vi "user process.vi"(8 "error in":errorcluster, 10 "MotionModule runtime in":refnum<class "MotionModule runtime.lvclass">, 11 "Parameters to process":T2) -> (0 "error out":errorcluster, 2 "MotionModule runtime Out":refnum<class "MotionModule runtime.lvclass">, 3 "Results from processing":T1)   [LabVIEW 2017, in "MotionModule runtime.lvclass"]
uses:
  MotionModule runtime.lvclass
  parameter user data.ctl
  result user data.ctl
  MotionModule runtime.lvclass/MotionModule runtime.ctl
  Utilities/StateMachine.ctl
  Utilities/Controlword_Commands.ctl
  Utilities/MoveMode.ctl
  SoftmotionClass/SoftmotionAxis/SoftmotionAxis.lvclass
  Utilities/WordManipulationLibrary.lvlib
  Utilities/Bit Manipulation.lvlib
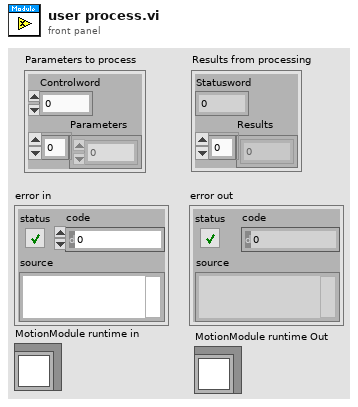
[diagram p1: front panel]
types:
  T1 = typedef "MotionModule runtime.lvclass/result user data.ctl" = cluster{"Statusword":u16, "Results":dbl[]}
  T2 = typedef "MotionModule runtime.lvclass/parameter user data.ctl" = cluster{"Controlword":u16, "Parameters":dbl[]}
  T3 = typedef "WordManipulationLibrary.lvlib/StateMachine.ctl" = enum16{"Start", "Not Ready to Switch On", "Switch On Disabled", "Ready to Switch On", "Switched On", "Operation enable", "Quick Stop Active", "Fault Reaction Active", "Fault"}
  T4 = typedef "WordManipulationLibrary.lvlib/Controlword_Commands.ctl" = enum16{"Shutdown", "Switch On", "Disable Voltage", "Quick Stop", "Disable Op", "Enable Op", "Fault Reset", "Error"}
  T5 = typedef "WordManipulationLibrary.lvlib/MoveMode.ctl" = enum16{"Reserved", "Profile Position Mode", "Velocity Mode", "Profile Velocity Mode", "Profile Torque Mode", "Reserved 2", "Reference Mode", "Interpolated Position Mode", "Skip"}
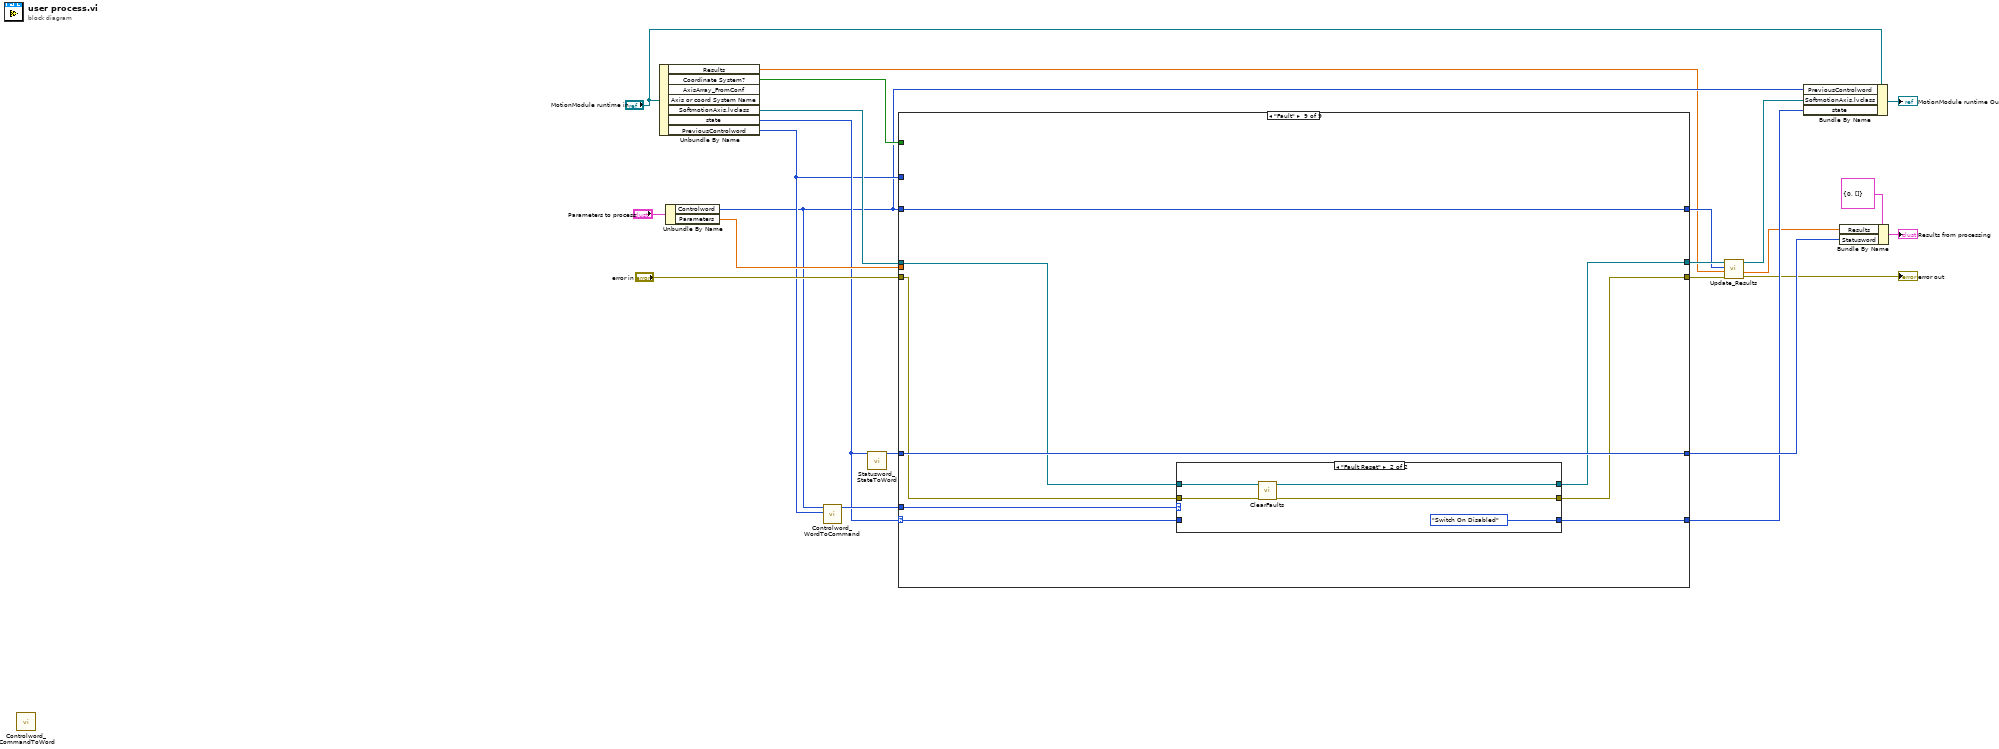
[diagram p0: block diagram]
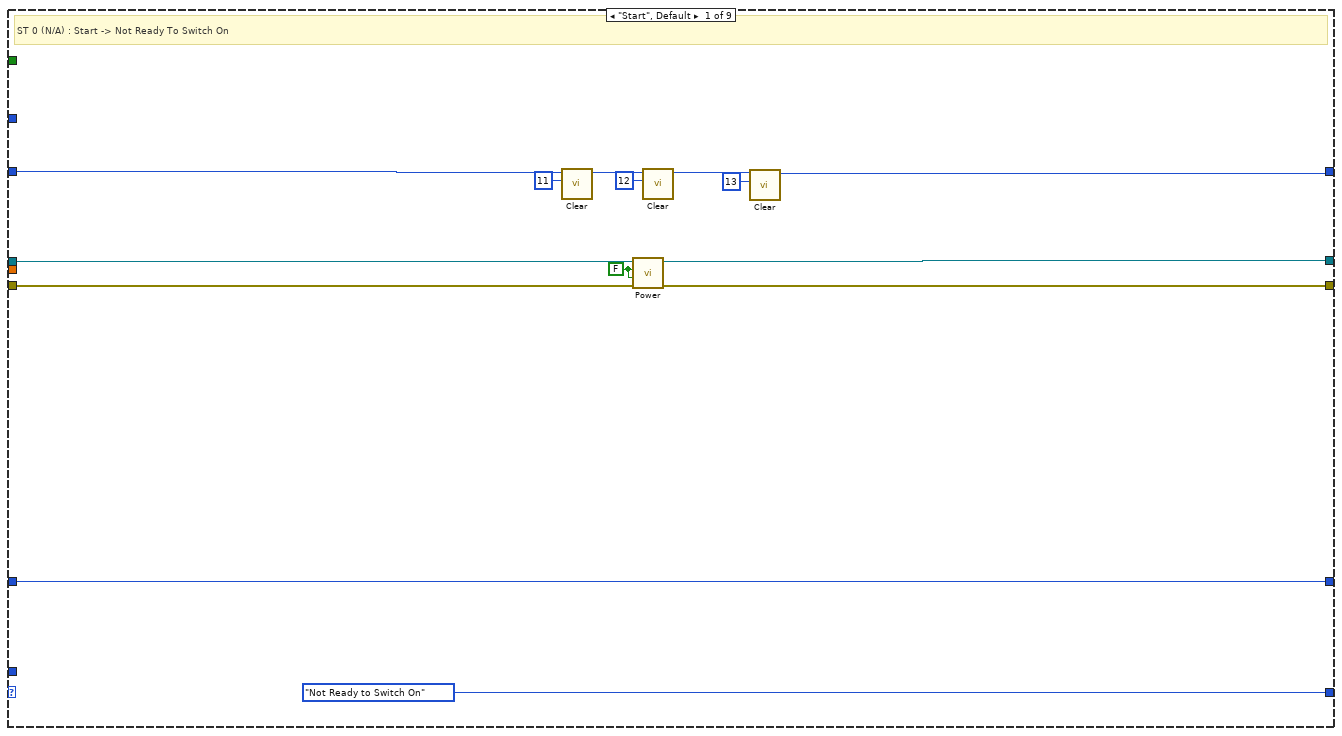
[diagram p2: hidden frame]
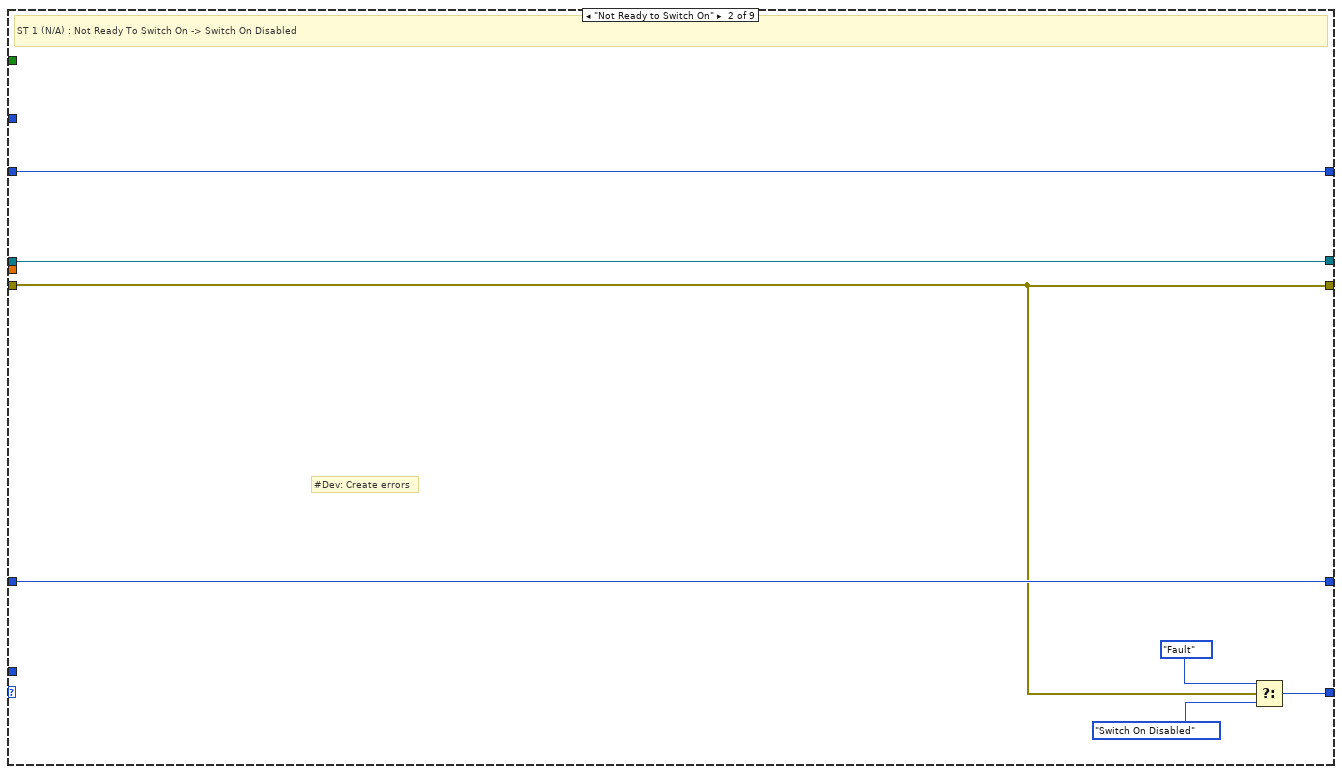
[diagram p3: hidden frame]
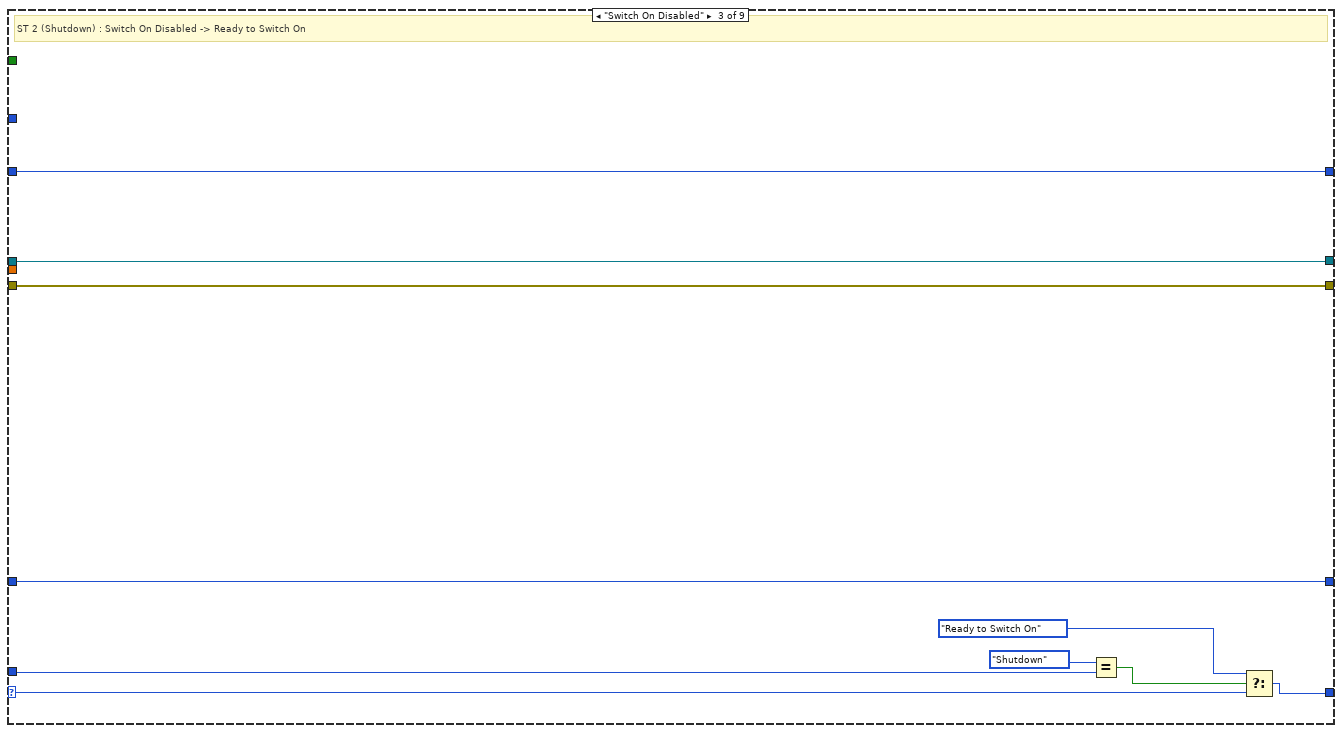
[diagram p4: hidden frame]
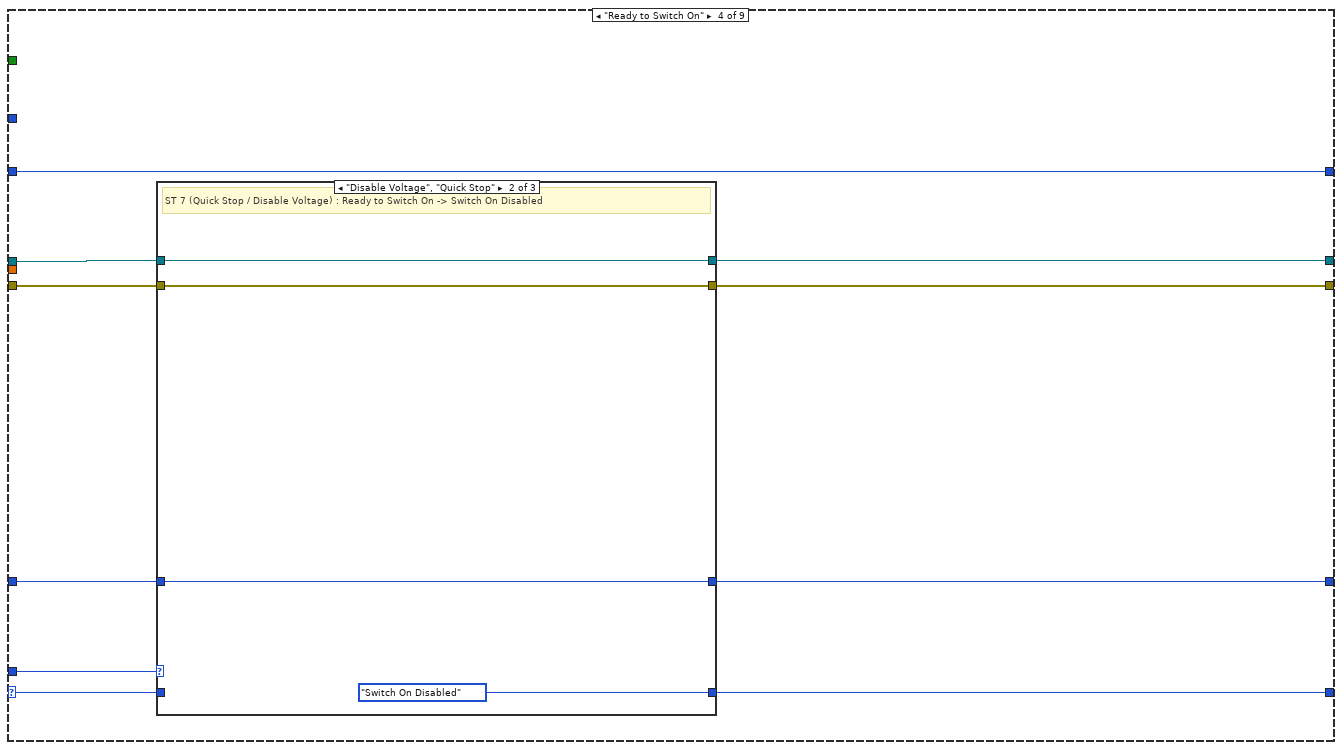
[diagram p5: hidden frame]
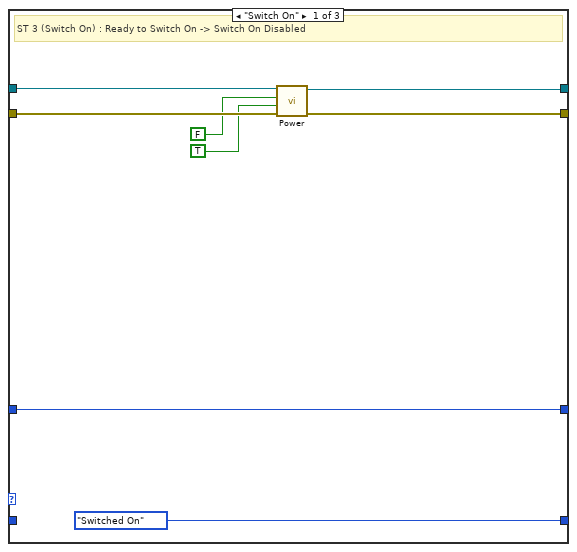
[diagram p6: hidden frame]
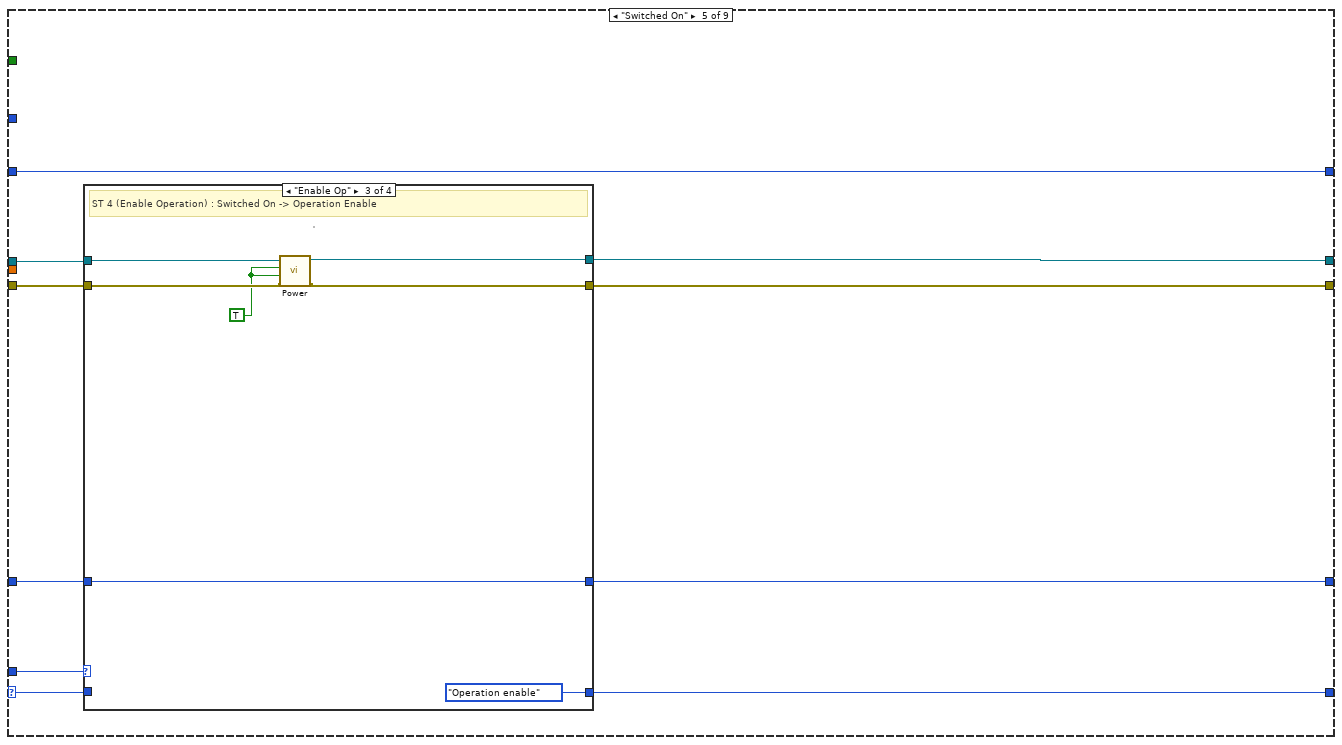
[diagram p8: hidden frame]
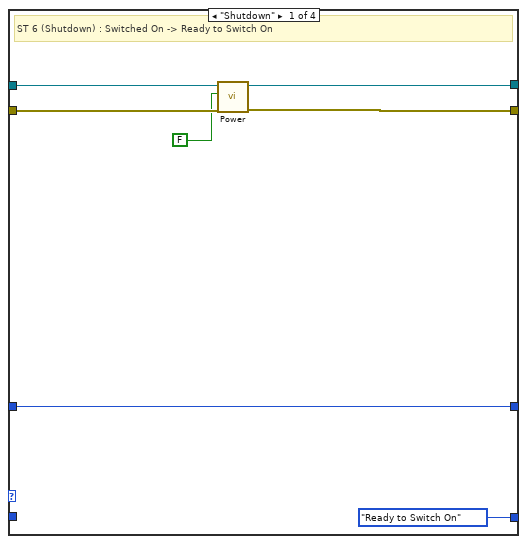
[diagram p9: hidden frame]
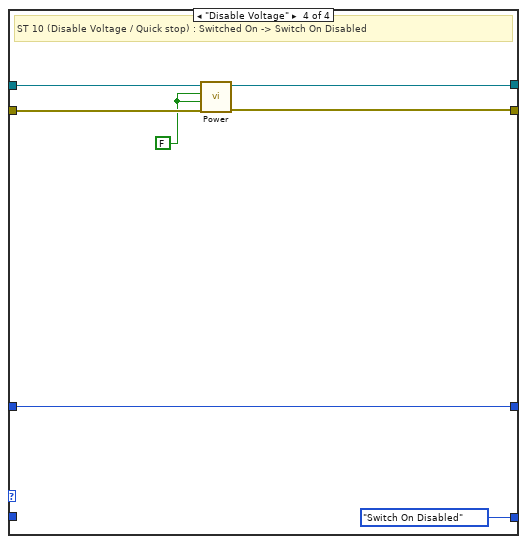
[diagram p11: hidden frame]
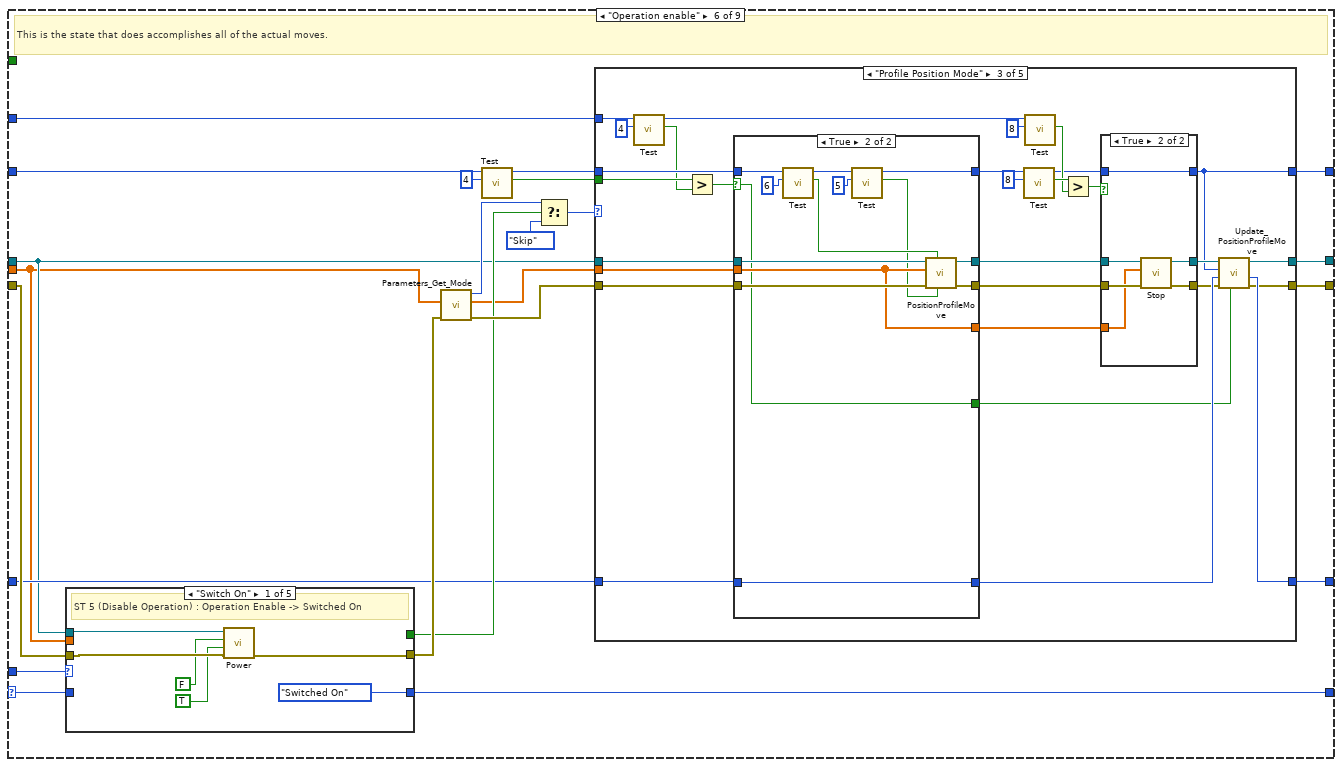
[diagram p12: hidden frame]
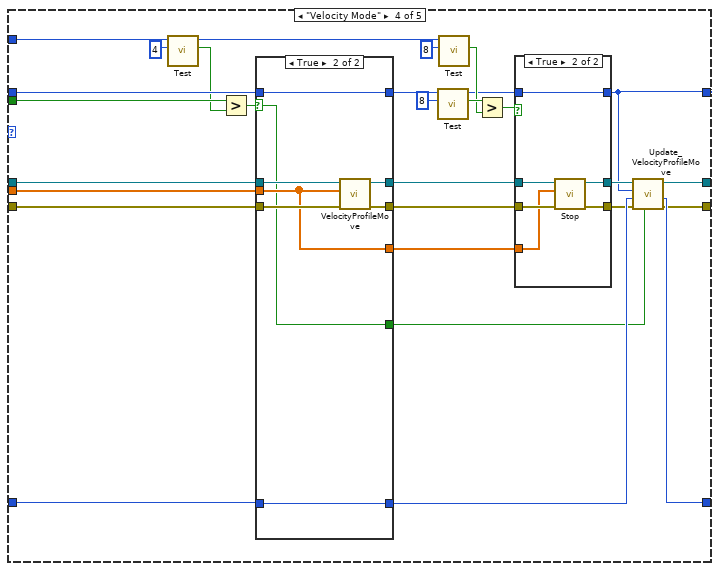
[diagram p17: hidden frame]
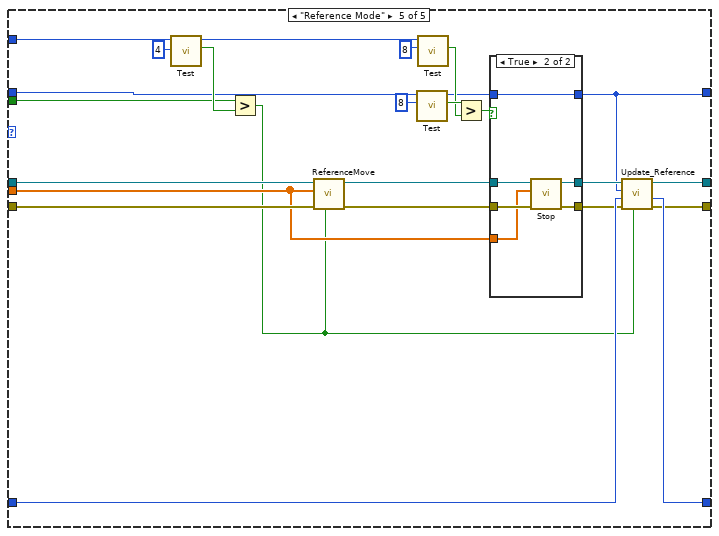
[diagram p20: hidden frame]
diagram:
  n1 = call "Controlword_CommandToWord.vi"() -> ()  [unwired: 11 in, 1 out]
  n2 = Unbundle By Name("MotionModule runtime in") -> ("Results"=w4:dbl[], "Coordinate System?"=w9:bool, "SoftmotionAxis.lvclass"=w18:refnum<class "SoftmotionAxis.lvclass">, "state"=w12:T3, "PreviousControlword"=w10:u16)  [unwired: 2 out]
  n3 = Unbundle By Name("Parameters to process") -> ("Controlword"=w8:u16, "Parameters"=w20:dbl[])
  n4 = call "Controlword_WordToCommand.vi"("Previous Controlword"=w10, "Controlword"=w8) -> ("Device Control Command"=w22:T4)  [unwired: 9 in]
  n5 = call "Statusword_StateToWord.vi"("CurrentStatus"=w12) -> ("StatusWord Out"=w23:u16)  [unwired: 10 in]
  n6 = case shown="\"Fault\"" w12 {
    selector: w12 -> [_ _ w50 w63 w89 w137 w319 _ w339]
    tunnel: w22 -> [_ _ w54 w64 w90 w138 w321 _ w340]
    tunnel: [StateMachine."Not Ready to Switch On" w41 w49 w62 w88 w118 w320 StateMachine."Fault" w341] -> w11
    tunnel: [w36 w44 w48 w58 w85 w134 w318 w331 w338] -> w13
    tunnel: w23 -> [w36 w44 w48 w59 w86 w124 w318 w331 w338]
    tunnel: w8 -> [w35 w38 w45 w55 w81 w136 w315 w325 w333]
    tunnel: w20 -> [_ _ _ _ _ w120 _ _ _]
    tunnel: "error in" -> [w26 w39 w47 w61 w87 w130 w316 w328 w337]
    tunnel: [w25 w39 w47 w60 w84 w119 w316 w327 w336] -> w7
    tunnel: w18 -> [w27 w40 w46 w57 w83 w122 w317 w330 w335]
    tunnel: [w24 w40 w46 w56 w82 w117 w317 w329 w334] -> w6
    tunnel: w10 -> [_ _ _ _ _ w121 _ _ _]
    tunnel: w9 -> [_ _ _ _ _ _ _ _ _]
    tunnel: [w29 w38 w45 w55 w81 w116 w315 w325 w333] -> w5
    frame "Start", Default {
      w28 = FALSE ("Enable Axis")
      # "ST 0 (N/A) : Start -> Not Ready To Switch On"
      n7 = call "Clear.vi"("Bit to clear"=u8 11, "Data_In"=w35) -> ("Data_Out"=w34:u16)  [unwired: 9 in]
      n8 = call-dynamic "Power.vi"("error in (no error)"=w26, "Enable Drive"=w28, "Enable Axis"=w28, "SoftmotionAxis in"=w27) -> ("error out"=w25:errorcluster, "SoftmotionAxis out"=w24:refnum<class "SoftmotionAxis.lvclass">)  [unwired: 6 in]
      n9 = call "Clear.vi"("Bit to clear"=u8 12, "Data_In"=w34) -> ("Data_Out"=w30:u16)  [unwired: 9 in]
      n10 = call "Clear.vi"("Bit to clear"=u8 13, "Data_In"=w30) -> ("Data_Out"=w29:u16)  [unwired: 9 in]
    }
    frame "Not Ready to Switch On" {
      # "#Dev: Create errors"
      # "ST 1 (N/A) : Not Ready To Switch On -> Switch On Disabled"
      n11 = Select(t=StateMachine."Fault", s=w39, f=StateMachine."Switch On Disabled") -> (s? t:f=w41:T3)
    }
    frame "Switch On Disabled" {
      # "ST 2 (Shutdown) : Switch On Disabled -> Ready to Switch On"
      n12 = Equal?(x=Controlword_Commands."Shutdown" ("Device Control Command"), y=w54) -> (x = y?=w53:bool)
      n13 = Select(t=StateMachine."Ready to Switch On", s=w53, f=w50) -> (s? t:f=w49:T3)
    }
    frame "Ready to Switch On" {
      n14 = case shown="\"Disable Voltage\", \"Quick Stop\"" w64 {
        tunnel: w63 -> [_ _ w80]
        tunnel: [StateMachine."Switched On" StateMachine."Switch On Disabled" w80] -> w62
        tunnel: w61 -> [w69 w75 w79]
        tunnel: [w70 w75 w79] -> w60
        tunnel: [w71 w74 w78] -> w58
        tunnel: w59 -> [w71 w74 w78]
        tunnel: w57 -> [w68 w73 w77]
        tunnel: [w65 w73 w77] -> w56
        frame "Switch On" {
          # "ST 3 (Switch On) : Ready to Switch On -> Switch On Disabled"
          n15 = call-dynamic "Power.vi"("error in (no error)"=w69, "Enable Drive"=TRUE, "Enable Axis"=FALSE, "SoftmotionAxis in"=w68) -> ("error out"=w70:errorcluster, "SoftmotionAxis out"=w65:refnum<class "SoftmotionAxis.lvclass">)  [unwired: 6 in]
        }
        frame "Disable Voltage", "Quick Stop" {
          # "ST 7 (Quick Stop / Disable Voltage) : Ready to Switch On -> Switch On Disabled"
        }
        frame Default {
          # "No Op."
        }
      }
    }
    frame "Switched On" {
      n16 = case shown="\"Enable Op\"" w90 {
        tunnel: w89 -> [_ w101 _ _]
        tunnel: [StateMachine."Ready to Switch On" w101 StateMachine."Operation enable" StateMachine."Switch On Disabled"] -> w88
        tunnel: w87 -> [w95 w100 w106 w113]
        tunnel: [w94 w100 w105 w112] -> w84
        tunnel: [w96 w99 w107 w114] -> w85
        tunnel: w86 -> [w96 w99 w107 w114]
        tunnel: w83 -> [w92 w98 w104 w111]
        tunnel: [w91 w98 w102 w110] -> w82
        frame "Shutdown" {
          # "ST 6 (Shutdown) : Switched On -> Ready to Switch On"
          n17 = call-dynamic "Power.vi"("error in (no error)"=w95, "Enable Axis"=FALSE, "SoftmotionAxis in"=w92) -> ("error out"=w94:errorcluster, "SoftmotionAxis out"=w91:refnum<class "SoftmotionAxis.lvclass">)  [unwired: 7 in]
        }
        frame Default {
          # "No op"
        }
        frame "Enable Op" {
          w103 = TRUE ("Enable Axis")
          # "ST 4 (Enable Operation) : Switched On -> Operation Enable"
          n18 = call-dynamic "Power.vi"("error in (no error)"=w106, "Enable Drive"=w103, "Enable Axis"=w103, "SoftmotionAxis in"=w104) -> ("error out"=w105:errorcluster, "SoftmotionAxis out"=w102:refnum<class "SoftmotionAxis.lvclass">)  [unwired: 6 in]
        }
        frame "Disable Voltage" {
          w109 = FALSE ("Enable Axis")
          # "ST 10 (Disable Voltage / Quick stop) : Switched On -> Switch On Disabled"
          n19 = call-dynamic "Power.vi"("error in (no error)"=w113, "Enable Drive"=w109, "Enable Axis"=w109, "SoftmotionAxis in"=w111) -> ("error out"=w112:errorcluster, "SoftmotionAxis out"=w110:refnum<class "SoftmotionAxis.lvclass">)  [unwired: 6 in]
        }
      }
    }
    frame "Operation enable" {
      # "This is the state that does accomplishes all of the actual moves."
      n20 = case shown="\"Switch On\"" w138 {
        tunnel: w137 -> [_ w299 _ _ _]
        tunnel: [StateMachine."Switched On" w299 StateMachine."Ready to Switch On" StateMachine."Switch On Disabled" StateMachine."Quick Stop Active"] -> w118
        tunnel: w130 -> [w295 w298 w303 w308 w313]
        tunnel: [w294 w298 w302 w307 w312] -> w129
        tunnel: [_ TRUE _ _ _] -> w126
        tunnel: w122 -> [w293 _ w300 w305 w311]
        tunnel: w120 -> [_ _ _ _ w310]
        frame "Switch On" {
          # "ST 5 (Disable Operation) : Operation Enable -> Switched On"
          n21 = call-dynamic "Power.vi"("error in (no error)"=w295, "Enable Drive"=TRUE, "Enable Axis"=FALSE, "SoftmotionAxis in"=w293) -> ("error out"=w294:errorcluster)  [unwired: 6 in, 1 out]
        }
        frame "Enable Op", Default {
        }
        frame "Shutdown" {
          w301 = FALSE ("Enable Axis")
          # "ST 8 (Shutdown) : Operation Enable -> Ready to Switch On"
          n22 = call-dynamic "Power.vi"("error in (no error)"=w303, "Enable Drive"=w301, "Enable Axis"=w301, "SoftmotionAxis in"=w300) -> ("error out"=w302:errorcluster)  [unwired: 6 in, 1 out]
        }
        frame "Disable Voltage" {
          w306 = FALSE ("Enable Axis")
          # "ST 9 (Disable Voltage) : Operation Enable -> Switch On Disabled"
          n23 = call-dynamic "Power.vi"("error in (no error)"=w308, "Enable Drive"=w306, "Enable Axis"=w306, "SoftmotionAxis in"=w305) -> ("error out"=w307:errorcluster)  [unwired: 6 in, 1 out]
        }
        frame "Quick Stop" {
          # "ST 11 (Quick Stop) : Operation Enable -> Quick Stop Active"
          n24 = call-dynamic "Stop.vi"("error in (no error)"=w313, "Parameters"=w310, "SoftmotionAxis in"=w311) -> ("error out"=w312:errorcluster)  [unwired: 7 in, 1 out]
        }
      }
      n25 = call "Parameters_Get_Mode.vi"("error in (no error)"=w129, "Parameters"=w120) -> ("error out"=w131:errorcluster, "Parameters Out"=w123:dbl[], "Move Mode"=w128:T5)  [unwired: 7 in]
      n26 = call "Test.vi"("Bit to test"=u8 4, "Data_In"=w136) -> ("bit value"=w132:bool, "Data_Out"=w133:u16)  [unwired: 8 in]
      n27 = Select(t=w128, s=w126, f=MoveMode."Skip") -> (s? t:f=w127:T5)
      n28 = case shown="\"Profile Position Mode\"" w127 {
        tunnel: w132 -> [_ _ w172 w230 w274]
        tunnel: [w142 w146 w168 w226 w278] -> w134
        tunnel: w124 -> [w142 w146 w171 w229 w279]
        tunnel: w133 -> [w139 w143 w175 w233 w266]
        tunnel: w123 -> [_ _ w173 w231 w261]
        tunnel: w131 -> [w141 w144 w174 w232 w280]
        tunnel: [w141 w144 w147 w206 w260] -> w119
        tunnel: w122 -> [w140 w145 w170 w228 w281]
        tunnel: [w140 w145 w148 w207 w259] -> w117
        tunnel: w121 -> [_ _ w166 w224 w275]
        tunnel: [w139 w143 w149 w205 w258] -> w116
        frame "Reserved", Default {
        }
        frame "Skip" {
        }
        frame "Profile Position Mode" {
          n29 = call "Test.vi"("Bit to test"=u8 4, "Data_In"=w166) -> ("bit value"=w165:bool, "Data_Out"=w156:u16)  [unwired: 8 in]
          n30 = Greater?(x=w172, y=w165) -> (0:w150:bool)
          n31 = case shown="True" w150 {
            selector: w150 -> [w185 w195]
            tunnel: w175 -> [w190 w204]
            tunnel: w174 -> [w188 w202]
            tunnel: w173 -> [w186 w196]
            tunnel: w171 -> [w187 w197]
            tunnel: w170 -> [w189 w200]
            tunnel: [w189 w199] -> w160
            tunnel: [w188 w198] -> w163
            tunnel: [w190 w193] -> w164
            tunnel: [w187 w197] -> w169
            tunnel: [w186 w196] -> w153
            tunnel: [w185 w195] -> w152
            frame False {
            }
            frame True {
              n32 = call "Test.vi"("Bit to test"=u8 6, "Data_In"=w204) -> ("bit value"=w201:bool, "Data_Out"=w194:u16)  [unwired: 8 in]
              n33 = call "Test.vi"("Bit to test"=u8 5, "Data_In"=w194) -> ("bit value"=w191:bool, "Data_Out"=w193:u16)  [unwired: 8 in]
              n34 = call-dynamic "PositionProfileMove.vi"("Immediate?"=w191, "Relative?"=w201, "error in (no error)"=w202, "Array"=w196, "SoftmotionAxis in"=w200) -> ("error out"=w198:errorcluster, "SoftmotionAxis out"=w199:refnum<class "SoftmotionAxis.lvclass">)  [unwired: 5 in]
            }
          }
          n35 = call "Test.vi"("Bit to test"=u8 8, "Data_In"=w164) -> ("bit value"=w158:bool, "Data_Out"=w154:u16)  [unwired: 8 in]
          n36 = call "Test.vi"("Bit to test"=u8 8, "Data_In"=w156) -> ("bit value"=w155:bool)  [unwired: 8 in, 1 out]
          n37 = Greater?(x=w158, y=w155) -> (0:w151:bool)
          n38 = case shown="True" w151 {
            tunnel: w163 -> [w178 w184]
            tunnel: [w178 w183] -> w162
            tunnel: [w177 w182] -> w161
            tunnel: w160 -> [w177 w181]
            tunnel: w154 -> [w176 w180]
            tunnel: [w176 w180] -> w149
            tunnel: w153 -> [_ w179]
            frame False {
            }
            frame True {
              n39 = call-dynamic "Stop.vi"("error in (no error)"=w184, "Parameters"=w179, "SoftmotionAxis in"=w181) -> ("error out"=w183:errorcluster, "SoftmotionAxis out"=w182:refnum<class "SoftmotionAxis.lvclass">)  [unwired: 7 in]
            }
          }
          n40 = call-dynamic "Update_PositionProfileMove.vi"("Skip Update?"=w152, "error in (no error)"=w162, "StatusWord"=w169, "ControlWord"=w149, "SoftmotionAxis in"=w161) -> ("error out"=w147:errorcluster, "StatusWord Out"=w168:u16, "SoftmotionAxis out"=w148:refnum<class "SoftmotionAxis.lvclass">)  [unwired: 4 in]
        }
        frame "Velocity Mode" {
          n41 = call "Test.vi"("Bit to test"=u8 4, "Data_In"=w224) -> ("bit value"=w223:bool, "Data_Out"=w214:u16)  [unwired: 8 in]
          n42 = Greater?(x=w230, y=w223) -> (0:w208:bool)
          n43 = case shown="True" w208 {
            selector: w208 -> [w243 w250]
            tunnel: w233 -> [w248 w249]
            tunnel: w232 -> [w246 w256]
            tunnel: w231 -> [w244 w251]
            tunnel: w229 -> [w245 w252]
            tunnel: w228 -> [w247 w255]
            tunnel: [w247 w254] -> w218
            tunnel: [w246 w253] -> w221
            tunnel: [w248 w249] -> w222
            tunnel: [w245 w252] -> w227
            tunnel: [w244 w251] -> w211
            tunnel: [w243 w250] -> w210
            frame False {
            }
            frame True {
              n44 = call-dynamic "VelocityProfileMove.vi"("error in (no error)"=w256, "Array"=w251, "SoftmotionAxis in"=w255) -> ("error out"=w253:errorcluster, "SoftmotionAxis out"=w254:refnum<class "SoftmotionAxis.lvclass">)  [unwired: 7 in]
            }
          }
          n45 = call "Test.vi"("Bit to test"=u8 8, "Data_In"=w222) -> ("bit value"=w216:bool, "Data_Out"=w212:u16)  [unwired: 8 in]
          n46 = call "Test.vi"("Bit to test"=u8 8, "Data_In"=w214) -> ("bit value"=w213:bool)  [unwired: 8 in, 1 out]
          n47 = Greater?(x=w216, y=w213) -> (0:w209:bool)
          n48 = case shown="True" w209 {
            tunnel: w221 -> [w236 w242]
            tunnel: [w236 w241] -> w220
            tunnel: [w235 w240] -> w219
            tunnel: w218 -> [w235 w239]
            tunnel: w212 -> [w234 w238]
            tunnel: [w234 w238] -> w205
            tunnel: w211 -> [_ w237]
            frame False {
            }
            frame True {
              n49 = call-dynamic "Stop.vi"("error in (no error)"=w242, "Parameters"=w237, "SoftmotionAxis in"=w239) -> ("error out"=w241:errorcluster, "SoftmotionAxis out"=w240:refnum<class "SoftmotionAxis.lvclass">)  [unwired: 7 in]
            }
          }
          n50 = call "Update_VelocityProfileMove.vi"("Skip Update?"=w210, "error in (no error)"=w220, "StatusWord"=w227, "ControlWord"=w205, "SoftmotionAxis in"=w219) -> ("error out"=w206:errorcluster, "StatusWord Out"=w226:u16, "SoftmotionAxis out"=w207:refnum<class "SoftmotionAxis.lvclass">)  [unwired: 4 in]
        }
        frame "Reference Mode" {
          n51 = call "Test.vi"("Bit to test"=u8 4, "Data_In"=w275) -> ("bit value"=w277:bool, "Data_Out"=w267:u16)  [unwired: 8 in]
          n52 = Greater?(x=w274, y=w277) -> (0:w257:bool)
          n53 = call-dynamic "ReferenceMove.vi"("New command"=w257, "error in (no error)"=w280, "Array"=w261, "SoftmotionAxis in"=w281) -> ("error out"=w262:errorcluster, "SoftmotionAxis out"=w263:refnum<class "SoftmotionAxis.lvclass">)  [unwired: 6 in]
          n54 = call "Test.vi"("Bit to test"=u8 8, "Data_In"=w266) -> ("bit value"=w272:bool, "Data_Out"=w268:u16)  [unwired: 8 in]
          n55 = call "Test.vi"("Bit to test"=u8 8, "Data_In"=w267) -> ("bit value"=w270:bool)  [unwired: 8 in, 1 out]
          n56 = Greater?(x=w272, y=w270) -> (0:w269:bool)
          n57 = case shown="True" w269 {
            tunnel: w262 -> [w284 w290]
            tunnel: [w284 w289] -> w264
            tunnel: [w283 w288] -> w265
            tunnel: w263 -> [w283 w287]
            tunnel: w268 -> [w282 w286]
            tunnel: [w282 w286] -> w258
            tunnel: w261 -> [_ w285]
            frame False {
            }
            frame True {
              n58 = call-dynamic "Stop.vi"("error in (no error)"=w290, "Parameters"=w285, "SoftmotionAxis in"=w287) -> ("error out"=w289:errorcluster, "SoftmotionAxis out"=w288:refnum<class "SoftmotionAxis.lvclass">)  [unwired: 7 in]
            }
          }
          n59 = call "Update_Reference.vi"("New Command"=w257, "error in (no error)"=w264, "StatusWord"=w279, "ControlWord"=w258, "SoftmotionAxis in"=w265) -> ("error out"=w260:errorcluster, "StatusWord Out"=w278:u16, "SoftmotionAxis out"=w259:refnum<class "SoftmotionAxis.lvclass">)  [unwired: 4 in]
        }
      }
    }
    frame "Quick Stop Active" {
      n60 = case shown="\"Shutdown\", Default" w321 {
        tunnel: w319 -> [_ _ w324]
        tunnel: [StateMachine."Operation enable" StateMachine."Switch On Disabled" w324] -> w320
        frame "Enable Op" {
          # "ST 16 (Enable Operation) : Quick Stop Active -> Operation Enable"
        }
        frame "Disable Voltage" {
          # "ST 12 (Quick Stop / Disable Voltage) : Quick Stop Active -> Switch On Disabled"
        }
        frame "Shutdown", Default {
          # "No Transition"
        }
      }
    }
    frame "Fault Reaction Active" {
      w326 = FALSE ("Enable Axis")
      # "#Dev: Deal with Fault here (Log, communicate, etc)"
      # "ST 14 (N/A) : Fault Reaction Active -> Fault"
      n61 = call-dynamic "Power.vi"("error in (no error)"=w328, "Enable Drive"=w326, "Enable Axis"=w326, "SoftmotionAxis in"=w330) -> ("error out"=w327:errorcluster, "SoftmotionAxis out"=w329:refnum<class "SoftmotionAxis.lvclass">)  [unwired: 6 in]
    }
    frame "Fault" {
      n62 = case shown="\"Fault Reset\"" w340 {
        tunnel: [w344 StateMachine."Switch On Disabled"] -> w341
        tunnel: w339 -> [w344 _]
        tunnel: w335 -> [w342 w348]
        tunnel: w337 -> [w343 w347]
        tunnel: [w343 w346] -> w336
        tunnel: [w342 w345] -> w334
        frame "Shutdown", Default {
        }
        frame "Fault Reset" {
          n63 = call-dynamic "ClearFaults.vi"("error in (no error)"=w347, "SoftmotionAxis in"=w348) -> ("error out"=w346:errorcluster, "SoftmotionAxis out"=w345:refnum<class "SoftmotionAxis.lvclass">)  [unwired: 8 in]
        }
      }
    }
  }
  n64 = call-dynamic "Update_Results.vi"("error in (no error)"=w7, "Results Array In"=w4, "ControlWord In"=w5, "SoftmotionAxis in"=w6) -> ("error out"=→"error out":errorcluster, "appended array"=w2:dbl[], "SoftmotionAxis out"=w3:refnum<class "SoftmotionAxis.lvclass">)  [unwired: 5 in]
  n65 = Bundle By Name(cluster="MotionModule runtime in", "PreviousControlword"=w8, "SoftmotionAxis.lvclass"=w3, "state"=w11) -> (→"MotionModule runtime Out":refnum<class "MotionModule runtime.lvclass">)
  n66 = Bundle By Name(cluster=T1 {"Statusword"=0, "Results"=[]} ("Results from processing"), "Results"=w2, "Statusword"=w13) -> (→"Results from processing":T1)
